vi "Read Data Configuration.vi"(8 "error in (no error)":errorcluster, 11 "CIF_Iceoryx_BB in":refnum<class "CIF_Iceoryx_BB.lvclass">) -> (0 "error out":errorcluster, 2 "Data Configuration":T1, 3 "CIF_Iceoryx_BB out":refnum<class "CIF_Iceoryx_BB.lvclass">)   [LabVIEW 2021, in "CIF_Iceoryx_BB.lvclass"]
uses:
  CIF_Iceoryx_BB.lvclass
  CIF_Iceoryx_BB.lvclass/CIF_Iceoryx_BB.ctl
  Typedef/Data Configuration.ctl
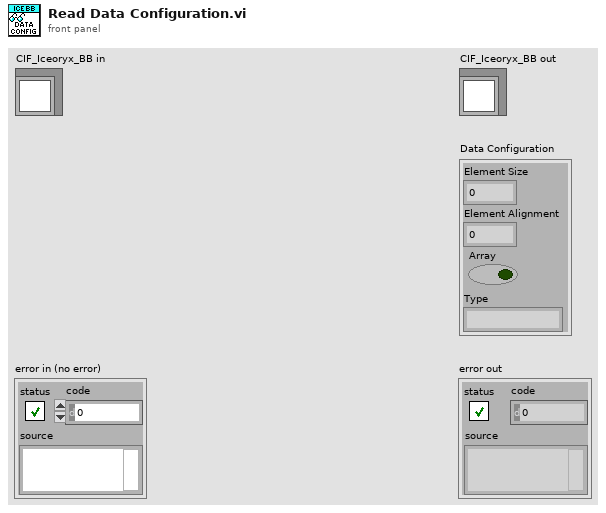
[diagram p1: front panel]
types:
  T1 = typedef "CIF_Iceoryx_BB.lvclass/Data Configuration.ctl" = cluster{"Element Size":u32, "Element Alignment":u32, "Array":bool, "Type":string}
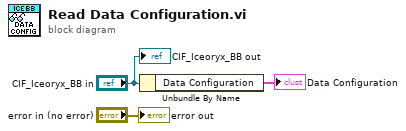
[diagram p0: block diagram]
diagram:
  n1 = Unbundle By Name("CIF_Iceoryx_BB in") -> ("Data Configuration"=→"Data Configuration":T1)
  "error out" <- "error in (no error)"
  "CIF_Iceoryx_BB out" <- "CIF_Iceoryx_BB in"
